vi "Release Memory Data.vi"(8 "error in (no error)":errorcluster caption="错误输入（无错误）", 11 "ptrData":T1) -> (0 "error out":errorcluster caption="错误输出", 1 "function return":i32, 2 "ptrData":string, 3 "ptrData out":T1)   [LabVIEW 2017, in "smncsftmt.lvlib"]
doc: "__declspec(dllexport) int ReleaseMemoryData(FtmtRawData* ptrData);"
uses:
  <vilib>/Utility/importsl/GetValueByPointer/datatype.ctl
  <vilib>/Utility/importsl/GetValueByPointer/GetValueByPointer.xnode
  smncsftmt.lvlib
  smncsftmt.dll
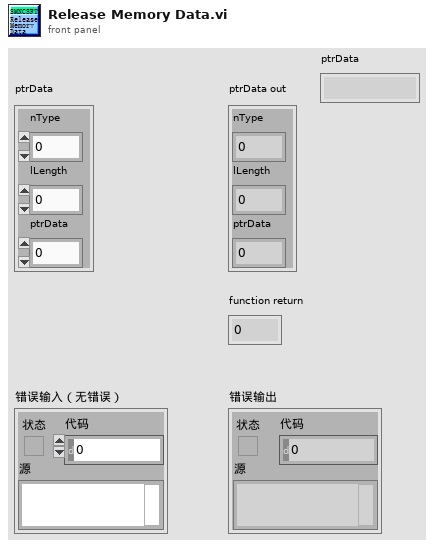
[diagram p1: front panel]
types:
  T1 = cluster{"nType":i32, "lLength":i32, "ptrData":u32}
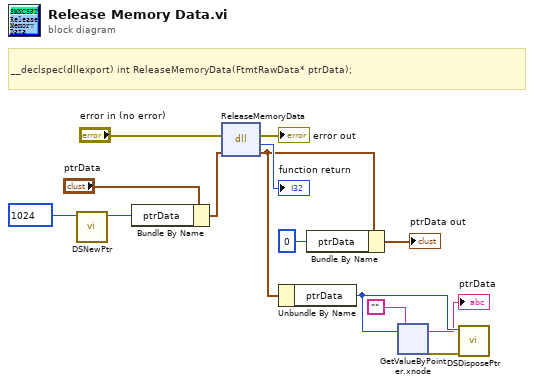
[diagram p0: block diagram]
diagram:
  # "__declspec(dllexport) int ReleaseMemoryData(FtmtRawData* ptrData);"
  n1 = call <vilib>:"DSNewPtr.vi"("Size"=u64 1024) -> ("Pointer"=w11:u64)  [unwired: 9 in, 1 out]
  n2 = Bundle By Name(cluster="ptrData", "ptrData"=w11) -> (w10:T1)
  n3 = dll-call lib="PTH2oabs CUsersaDesktop\nLABVIEW范例National InstrumentsLabVIEW 2017user.lib\tsmncsftmtsmncsftmt.*" fn="ReleaseMemoryData"(error in="error in (no error)", "ptrData"=w10) -> (error out=→"error out":errorcluster, →"function return":i32, "ptrData"=w5:T1)  [unwired: 2 in, 1 out]
  n4 = Unbundle By Name(w5) -> ("ptrData"=w8:u32)
  n5 = Bundle By Name(cluster=w5, "ptrData"=u32 0) -> (→"ptrData out":T1)
  n6 = xnode "GetValueByPointer.xnode"("Pointer"=w8, "InputType"="") -> ("Output"=→"ptrData":string, "ErrorOut"=w9:errorcluster)  [unwired: 2 in]
  n7 = call <vilib>:"DSDisposePtr.vi"("error in (no error)"=w9, "Pointer"=w8) -> ()  [unwired: 9 in, 1 out]
